vi "Voir compteurs.vi"() -> ()   [LabVIEW 2022 SP3]
uses:
  Enum/Enum compteur 4.ctl
  Variables globales/Variable globale compteurs.vi
panel:
  out "Temps débit":u16 caption="Temps pour calcul débit" format="%<%H:%M:%S>t"
  out "Noms":string[](array[string]) caption="Noms des compteurs sélectionnés"
  out "valeurs":dbl[](array[numeric]) format="%.2f"
  out "référence en sortie":refnum<vi>
  in  "stop":bool
  # "Valeurs\ncompteurs GN2"
  # "Ce logiciel et les informations qu'il contient, sont la propriété de l’IAS \net ne peuvent être diffusés sans l’autorisation de la Station d’étalonnage"
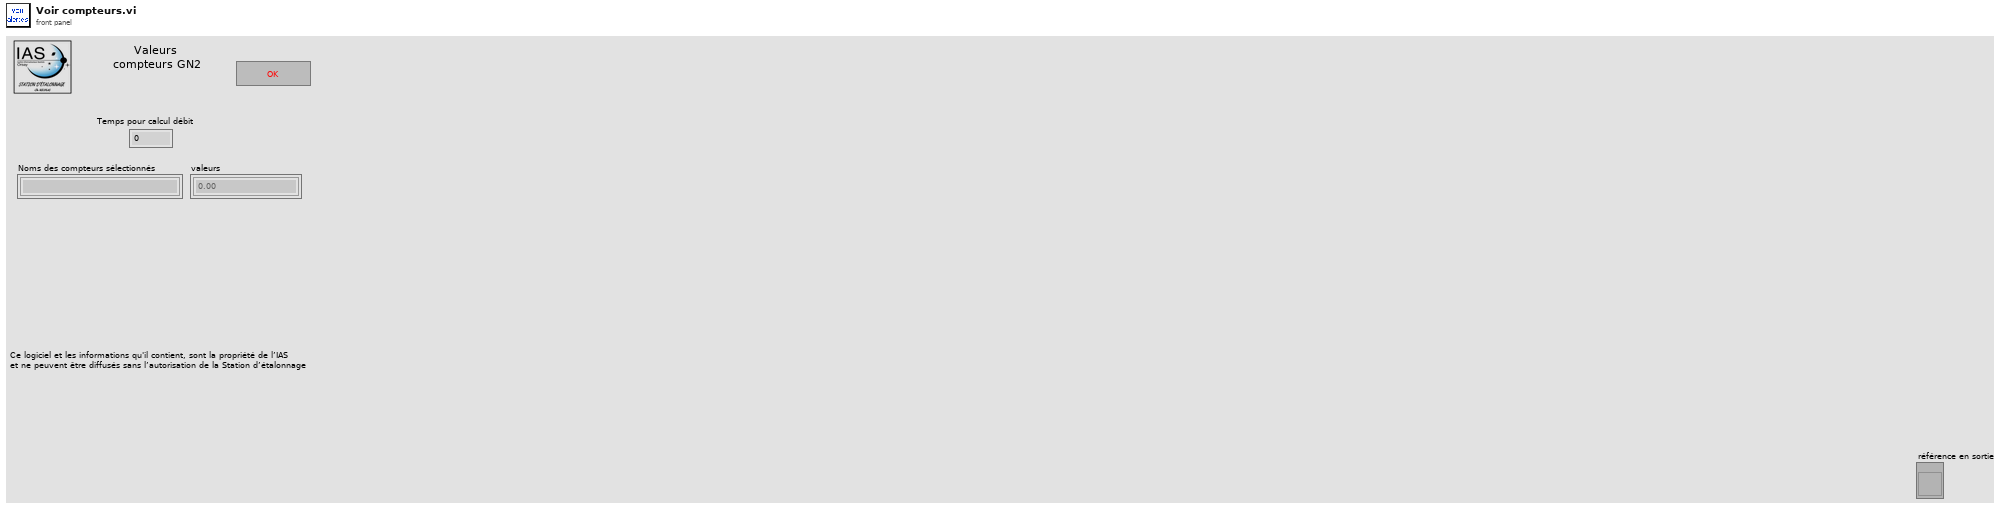
[diagram p1: front panel]
types:
  T1 = typedef "Enum compteur 4.ctl" = enum16{"init", "attente", "fin"}
  T2 = enum32{"Invalid", "Standard", "Closed", "Hidden", "Minimized", "Maximized"}
  T3 = cluster{"Nom tache compteurs":refnum<k21>, "Noms des compteurs":string[], "Selection":bool[], "Init compteurs":dbl[], "Noms compteurs selectionnes":string[]}
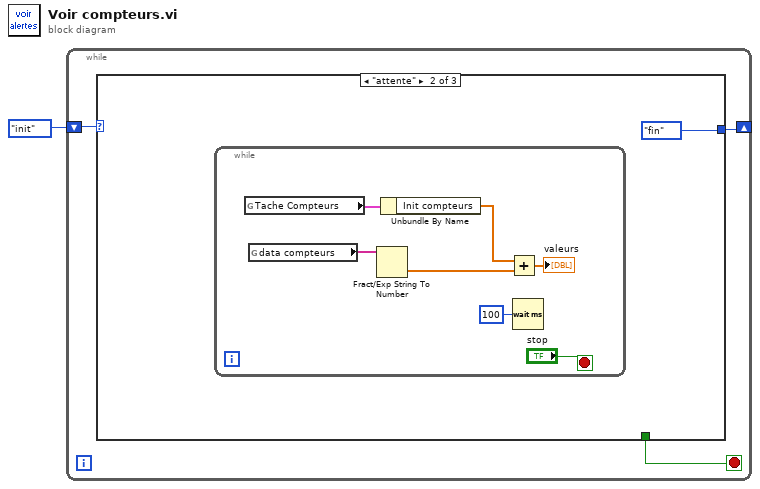
[diagram p0: block diagram]
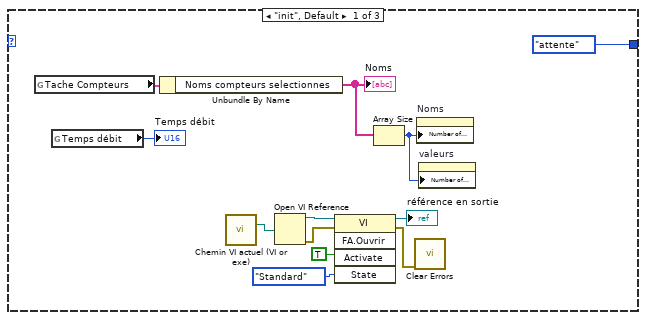
[diagram p2: hidden frame]
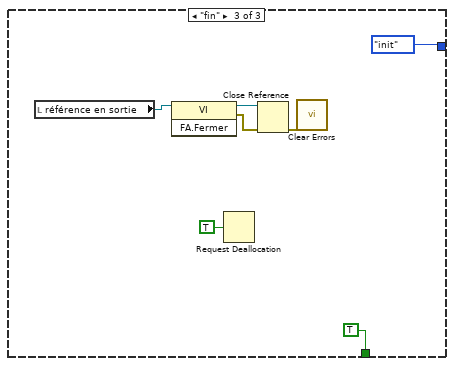
[diagram p3: hidden frame]
diagram:
  n1 = while {
    shift-right: [w3] -> _
    shift-left: Enum_compteur_4."init" ("Énum") -> [w4]
    stop <- w2 stop-if-true
    n2 = case shown="\"attente\"" w4 {
      tunnel: [Enum_compteur_4."attente" ("Énum") Enum_compteur_4."fin" ("Énum") Enum_compteur_4."init" ("Énum")] -> w3
      tunnel: [_ _ TRUE] -> w2
      frame "init", Default {
        n3 = global read "Variable globale compteurs.vi" "Tache Compteurs"() -> (w8:T3)
        n4 = global read "Variable globale compteurs.vi" "Temps débit"() -> (→"Temps débit":u16)
        n5 = Unbundle By Name(w8) -> ("Noms compteurs selectionnes"=w7:string[])
        "Noms" <- w7
        n6 = call "Chemin VI actuel (VI or exe).vi"() -> ("Full Path to VI or executable"=w9:path)  [unwired: 14 in, 1 out]
        n7 = Open VI Reference(vi path=w9) -> (vi reference=w13:refnum<vi>, error out=w15:errorcluster)  [unwired: 5 in]
        n8 = invoke class="VI" method="FA.Ouvrir"(reference=w13, error in=w15, "Activate"=TRUE ("Activer ?"), "State"=T2."Standard" ("État")) -> (reference out=→"référence en sortie":refnum<vi>, error out=w16:errorcluster)  [unwired: 1 in, 3 out]
        n9 = Array Size(array=w7) -> (size(s)=w6:i32)
        n10 = call <vilib>:"Clear Errors.vi"("error in (no error)"=w16) -> ()  [unwired: 5 in, 2 out]
        n11 = property on="Noms" class="Tabl (strict)"("Number of Rows"=w6) -> ()  [unwired: 2 in, 2 out]
        n12 = property on="valeurs" class="Tabl (strict)"("Number of Rows"=w6) -> ()  [unwired: 2 in, 2 out]
      }
      frame "attente" {
        n13 = while {
          stop <- "stop" stop-if-true
          n14 = global read "Variable globale compteurs.vi" "Tache Compteurs"() -> (w22:T3)
          n15 = global read "Variable globale compteurs.vi" "data compteurs"() -> (w21:string[])
          n16 = Fract/Exp String To Number(string=w21) -> (number=w19:dbl[])  [unwired: 3 in, 1 out]
          n17 = Unbundle By Name(w22) -> ("Init compteurs"=w20:dbl[])
          n18 = Add(x=w20, y=w19) -> (x+y=→"valeurs":dbl[])
          n19 = Wait (ms)(milliseconds to wait=u32 100 ("attente (ms)")) -> ()  [unwired: 1 out]
        }
      }
      frame "fin" {
        n20 = local read "référence en sortie"() -> (w25:refnum<vi>)
        n21 = invoke class="VI" method="FA.Fermer"(reference=w25) -> (reference out=w27:refnum<vi>, error out=w26:errorcluster)  [unwired: 2 in, 1 out]
        n22 = Request Deallocation(TRUE ("flag")) -> ()
        n23 = Close Reference(reference=w27, error in (no error)=w26) -> (error out=w28:errorcluster)
        n24 = call <vilib>:"Clear Errors.vi"("error in (no error)"=w28) -> ()  [unwired: 5 in, 2 out]
      }
    }
  }
